vi "LabVIEW CLI argument missing--error.vi"() -> (0 "error out":errorcluster)   [LabVIEW 2026]
doc: "This error signalizes that a required LabVIEW CLI argument is missing."
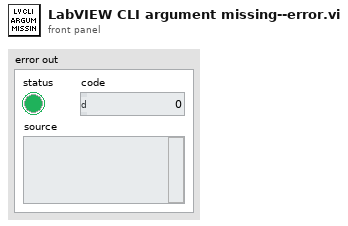
[diagram p1: front panel]
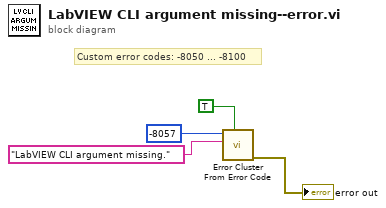
[diagram p0: block diagram]
diagram:
  # "Custom error codes: -8050 ... -8100"
  n1 = call <vilib>:"Error Cluster From Error Code.vi"("show call chain? (False)"=TRUE, "error message (\"\")"="LabVIEW CLI argument missing." ("error message (\"\")"), "error code (0)"=-8057) -> ("error out"=→"error out":errorcluster)  [unwired: 6 in]
